vi "Read XY Plotter.vi"(8 "error in (no error)":errorcluster, 11 "XY Plotter configuration in":refnum<class "XY Plotter configuration.lvclass">) -> (0 "error out":errorcluster, 2 "H1 Plotter Setting":T1={"Data Rate"=20, "Y-Scales"=[{"Label"="Amplitude", "Max"=5.0, "Min"=-5.0, "Unit"=enum."in", "Visible"=TRUE}, {"Label"="", "Max"=100.0, "Min"=-100.0, "Unit"=enum."---", "Visible"=TRUE}], "Note"="", "History Length"=5, "DataLog Path"=path "C:/_Data_Log", "Plot type"=FALSE, "X-Scales"=[{"Label"="Amplitude", "Max"=5.0, "Min"=-5.0, "Unit"=enum."in", "Visible"=TRUE}, {"Label"="", "Max"=100.0, "Min"=-100.0, "Unit"=enum."---", "Visible"=TRUE}], "Plot List"=[{"Plot Name"="Ch1", "X Scale Index"=0, "Y Scale Index"=0, "Visible"=TRUE}, {"Plot Name"="Ch1", "X Scale Index"=0, "Y Scale Index"=0, "Visible"=TRUE}]}, 3 "XY Plotter configuration out":refnum<class "XY Plotter configuration.lvclass">)   [LabVIEW 2025, in "XY Plotter.lvlib" / "XY Plotter configuration.lvclass"]
uses:
  XY Plotter configuration.lvclass
  XY Plotter.ctl
  XY Plotter configuration.lvclass/XY Plotter configuration.ctl
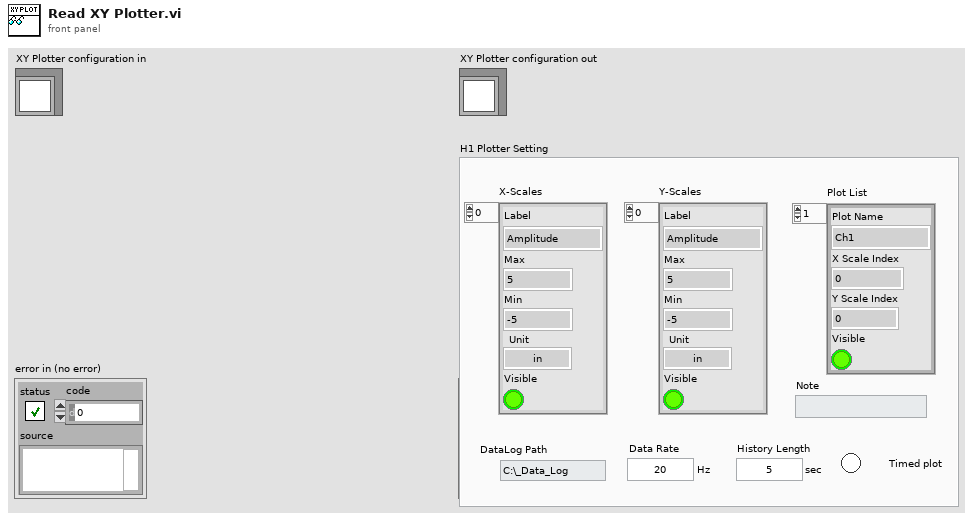
[diagram p1: front panel]
types:
  T1 = typedef "XY Plotter.lvlib/XY Plotter configuration.lvclass/XY Plotter.ctl" = cluster{"Data Rate":i32, "Y-Scales":cluster{"Label":string, "Max":dbl, "Min":dbl, "Unit":enum16{"---", "V", "mA", "sec", "dB", "deg", "in/s", "in", "lbf", "Hz", "psi", "gpm"}, "Visible":bool}[], "Note":string, "History Length":i32, "DataLog Path":path, "Plot type":bool, "X-Scales":cluster{"Label":string, "Max":dbl, "Min":dbl, "Unit":enum16{"---", "V", "mA", "sec", "dB", "deg", "in/s", "in", "lbf", "Hz", "psi", "gpm"}, "Visible":bool}[], "Plot List":cluster{"Plot Name":string, "X Scale Index":u32, "Y Scale Index":u32, "Visible":bool}[]}
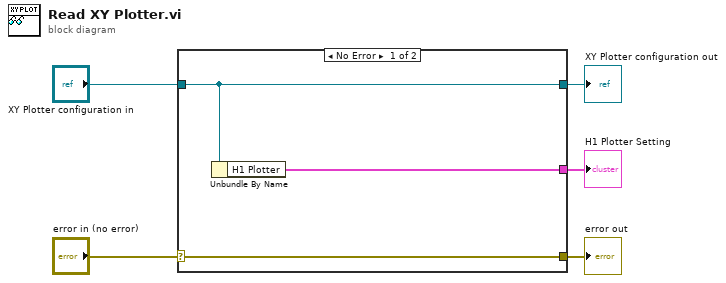
[diagram p0: block diagram]
diagram:
  n1 = case shown="No Error" "error in (no error)" {
    selector: "error in (no error)" -> [w8 w9]
    tunnel: [w8 w9] -> w4
    tunnel: [w7 w10] -> w2
    tunnel: "XY Plotter configuration in" -> [w7 w10]
    tunnel: [w6 _] -> w1
    frame No Error {
      n2 = Unbundle By Name(w7) -> ("H1 Plotter"=w6:T1)
    }
    frame Error {
    }
  }
  "error out" <- w4
  "XY Plotter configuration out" <- w2
  "H1 Plotter Setting" <- w1
